vi "RDC-saltwater-generate_perm.vi"(8 "Increment f (10MHz)":dbl=10000000.0, 9 "Stop f (6GHz) 2":dbl=6000000000.0, 10 "Start f (300MHz)":dbl=300000000.0, 11 "water Temp (25C) [10-40C]":dbl=25.0) -> (0 "used temp":dbl, 1 "Complex Perm":cluster{dbl[], cdb[]}, 2 "Imag Perm":cluster{dbl[], dbl[]}, 3 "Real Perm":cluster{dbl[], dbl[]}, 4 "Complex perm":cdb[](array[numeric]))   [LabVIEW 2020, in "RDC-Reflection_Data_Computation.lvlib"]
doc: "Generates the salt water model permittivity over a frequency range (start, stop, increment) at the given water temperature (10-40 C). Returns the complex, real and imaginary permittivity and the temperature used."
uses:
  RDC-Reflection_Data_Computation.lvlib
panel:
  out "unsigned 16bit integer":i32
  out "loss":cluster{dbl[], dbl[]}[](graph)
  out "perm":cluster{dbl[], dbl[]}[](graph)
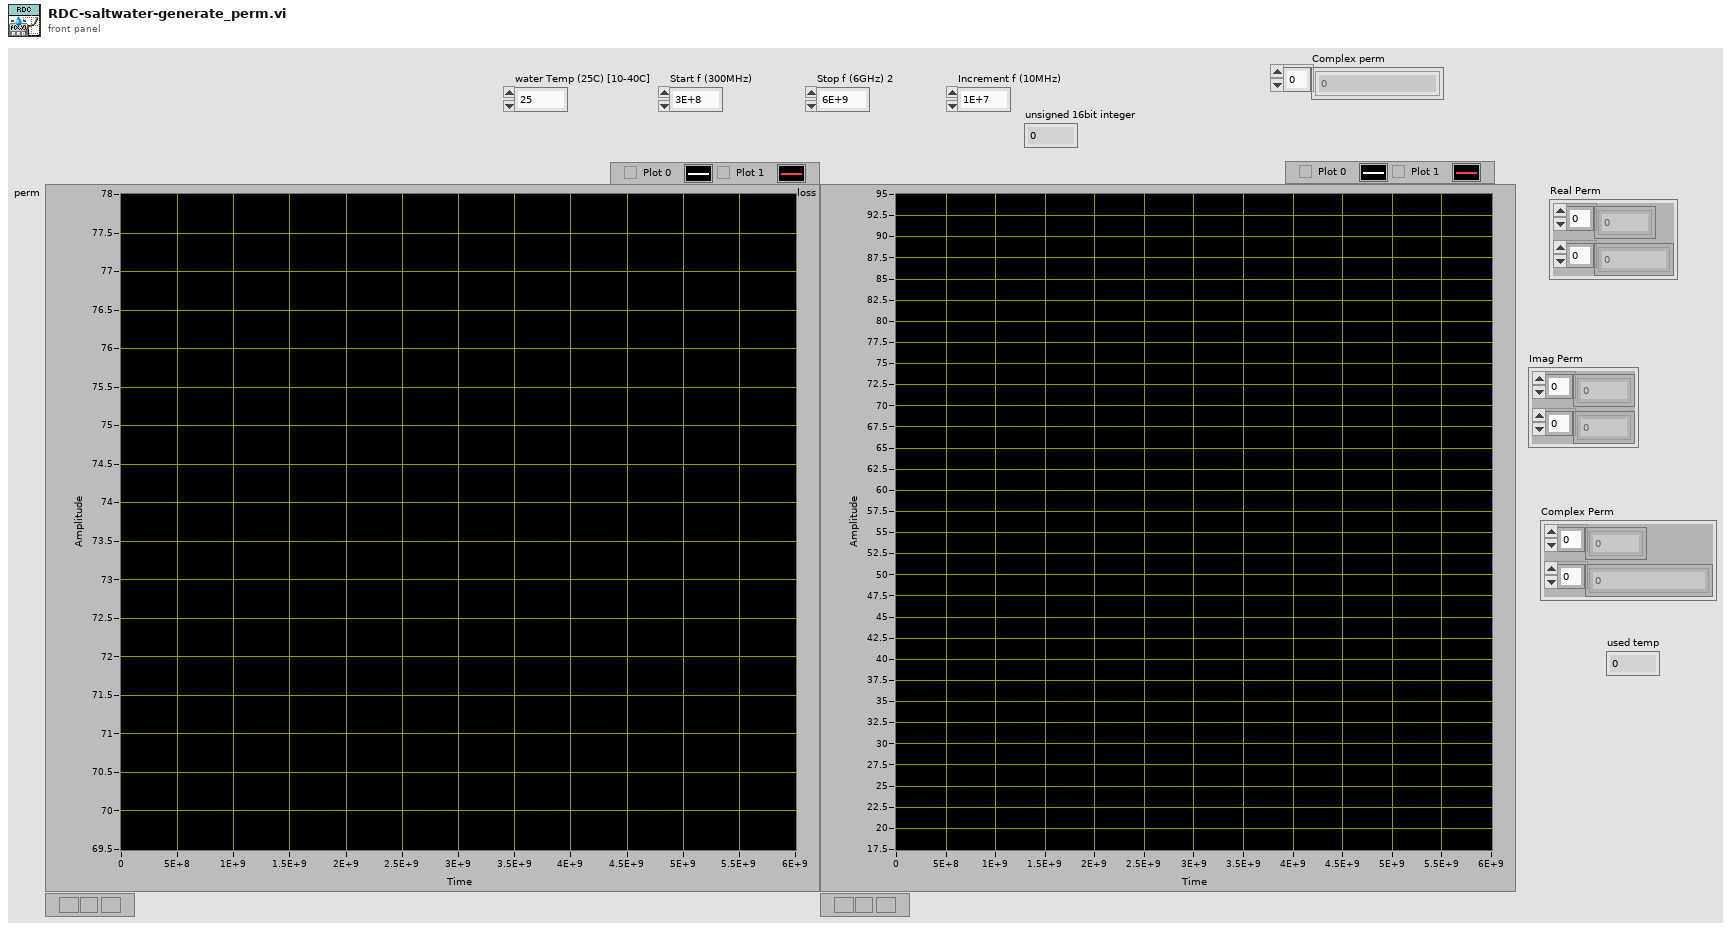
[diagram p1: front panel]
types:
  T1 = typedef "RDC-Reflection_Data_Computation.lvlib/RDC-saltwater-param.ctl" = cluster{"temp Cx10":u16, "eps s":dbl, "eps infi":dbl, "tau":dbl, "alpha":dbl, "sigma":dbl, "eps s diff":dbl, "eps infi diff":dbl, "tau diff":dbl, "alpha diff":dbl, "sigma diff":dbl}
  T2 = cluster{"Frequency":dbl[], "Reflection'":dbl[]}[]
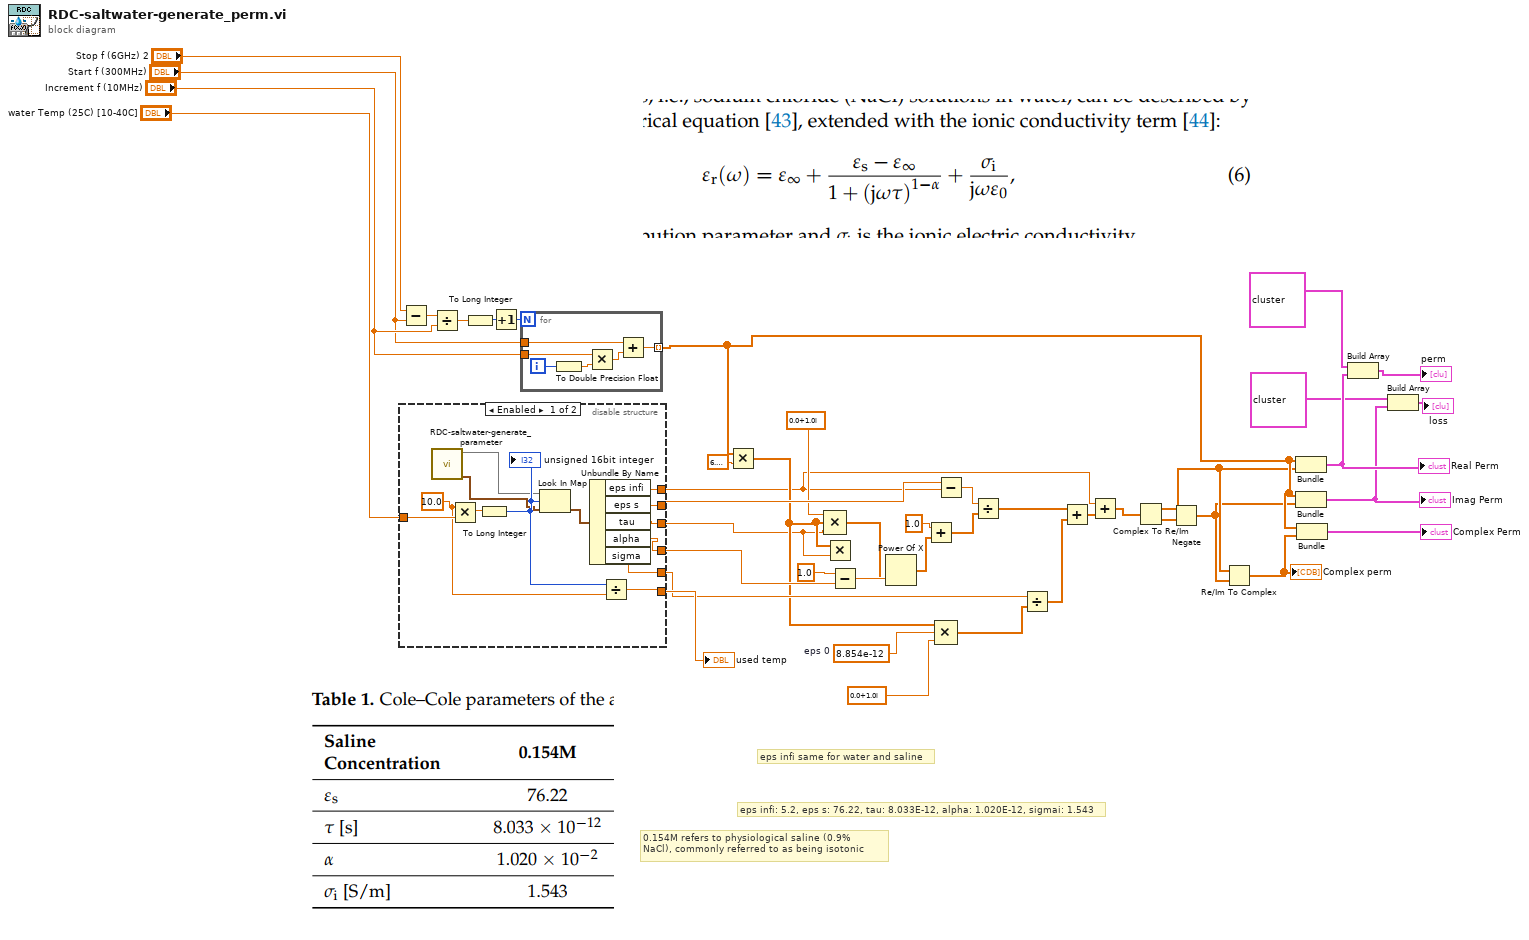
[diagram p0: block diagram]
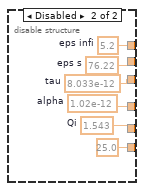
[diagram p2: hidden frame]
diagram:
  w17 = 8.854e-12  # eps 0
  # "eps infi: 5.2, eps s: 76.22, tau: 8.033E-12, alpha: 1.020E-12, sigmai: 1.543"
  # "0.154M refers to physiological saline (0.9%\nNaCl), commonly referred to as being isotonic"
  # "eps infi same for water and saline"
  n1 = disable-structure shown="Enabled" {
    disable-tunnel: "water Temp (25C) [10-40C]" -> [w56 _]
    disable-tunnel: [w53 w61] -> w33
    disable-tunnel: [w52 w62] -> w5
    disable-tunnel: [w51 w60] -> w14
    disable-tunnel: [w48 25.0 ("used temp")] -> w31
    disable-tunnel: [w46 w59] -> w29
    disable-tunnel: [w45 w57] -> w24
    frame Enabled {
      w49 = 10.0 ("x")
      n2 = call "RDC-saltwater-generate_parameter.vi"() -> ("defalut"=w44:T1, "map"=w47:map{i32, T1})  [unwired: 10 in]
      n3 = Multiply(x=w49, y=w56) -> (x*y=w55:dbl)
      n4 = To Long Integer(number=w55) -> (32bit integer=w50:i32)
      "unsigned 16bit integer" <- w50
      n5 = Look In Map(map=w47, key=w50, default value=w44) -> (value=w54:T1)  [unwired: 1 out]
      n6 = Unbundle By Name(w54) -> ("eps infi"=w52:dbl, "eps s"=w53:dbl, "tau"=w51:dbl, "alpha"=w46:dbl, "sigma"=w45:dbl)
      n7 = Divide(x=w50, y=w49) -> (x/y=w48:dbl)
    }
    frame Disabled {
      w59 = 1.02e-12  # alpha
      w57 = 1.543  # Qi
      w60 = 8.033e-12  # tau
      w61 = 76.22  # eps s
      w62 = 5.2  # eps infi
    }
  }
  "used temp" <- w31
  n8 = Subtract(x="Stop f (6GHz) 2", y="Start f (300MHz)") -> (x-y=w42:dbl)
  n9 = Divide(x=w42, y="Increment f (10MHz)") -> (x/y=w40:dbl)
  n10 = To Long Integer(number=w40) -> (32bit integer=w39:i32)
  n11 = Increment(x=w39) -> (x+1=w30:i32)
  n12 = for {
    N: w30 -> [_]
    tunnel: "Start f (300MHz)" -> [w66]
    tunnel: "Increment f (10MHz)" -> [w65]
    tunnel: [w63] -> w34 mode=indexing
    i -> [w64]
    n13 = To Double Precision Float(number=w64) -> (double precision float=w68:dbl)
    n14 = Multiply(x=w65, y=w68) -> (x*y=w67:dbl)
    n15 = Add(x=w66, y=w67) -> (x+y=w63:dbl)
  }
  n16 = Multiply(x=w34, y=6.283185307179586) -> (x*y=w15:dbl[])
  n17 = Compound Arithmetic op=MULTIPLY(cdb 0.0+1.0i ("y"), w15, w14) -> (w13:cdb[])
  n18 = Multiply(x=w15, y=w14) -> ()  [unwired: 1 out]
  n19 = Subtract(x=1.0, y=w29) -> (x-y=w28:dbl)
  n20 = Power Of X(1:w13, 2:w28) -> (0:w27:cdb[])
  n21 = Add(x=1.0, y=w27) -> (x+y=w26:cdb[])
  n22 = Compound Arithmetic op=MULTIPLY(w15, w17, cdb 0.0+1.0i ("y")) -> (w12:cdb[])
  n23 = Subtract(x=w33, y=w5) -> (x-y=w32:dbl)
  n24 = Divide(x=w32, y=w26) -> (x/y=w25:cdb[])
  n25 = Divide(x=w24, y=w12) -> (x/y=w23:cdb[])
  n26 = Add(x=w25, y=w23) -> (x+y=w6:cdb[])
  n27 = Add(x=w5, y=w6) -> (x+y=w4:cdb[])
  n28 = Complex To Re/Im(x + iy=w4) -> (x=w3:dbl[], y=w11:dbl[])
  n29 = Negate(x=w11) -> (-x=w2:dbl[])
  n30 = Re/Im To Complex(1:w2, 2:w3) -> (0:w1:cdb[])
  "Complex perm" <- w1
  n31 = Bundle(w34, w3) -> (w19:cluster{dbl[], dbl[]})  [unwired: 1 in]
  "Real Perm" <- w19
  n32 = Bundle(w34, w2) -> (w18:cluster{dbl[], dbl[]})  [unwired: 1 in]
  "Imag Perm" <- w18
  n33 = Bundle(w34, w1) -> (→"Complex Perm":cluster{dbl[], cdb[]})  [unwired: 1 in]
  n34 = Build Array(cluster{"Frequency":dbl[], "Reflection'":dbl[]} {"Frequency"=array[2001 elements], "Reflection'"=array[2001 elements]} ("element 2"), w19) -> (→"perm":T2)
  n35 = Build Array(cluster{"Frequency":dbl[], "Reflection'":dbl[]} {"Frequency"=array[2001 elements], "Reflection'"=array[2001 elements]} ("element"), w18) -> (→"loss":T2)
